vi "MQTT Session - Get Maximum QoS.vi"(0 "MQTT Session":T2, 7 "QoS":T1, 11 "error in":errorcluster) -> (4 "MQTT Session Out":T2, 8 "QoS":T1, 15 "error out":errorcluster)   [LabVIEW 2019, in "KoRE-MQTT.lvlib"]
doc: "Copyright (c) 2025 KoRElibs.com\nSPDX-License-Identifier: EUPL-1.2\n\nThis VI is licensed under the European Union Public License (EUPL) Version 1.2. You may use this VI unmodified in proprietary works. If you distribute a modified version of this file, the modified file must be released under the EUPL-1.2. Full license: https://joinup.ec.europa.eu/asset/eupl/eupl/1.2/"
uses:
  KoRE-MQTT.lvlib
  Public/TypeDefs/MQTT QoS Level.ctl
  Public/TypeDefs/MQTT Client Session.ctl
  TypeDefs/MQTT Client Session - Data Value Reference.ctl
  Public/TypeDefs/MQTT Client Session - Data.ctl
  Public/TypeDefs/MQTT Property - Will.ctl
  Public/TypeDefs/MQTT Property - CONNECT.ctl
  TypeDefs/MQTT Subscription - Info.ctl
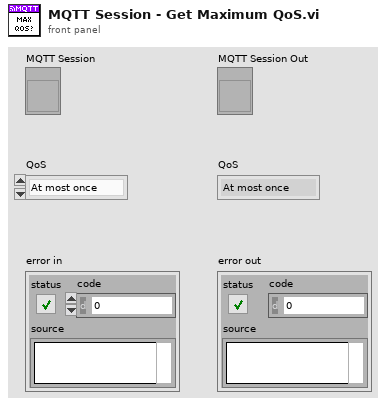
[diagram p1: front panel]
types:
  T1 = typedef "KoRE-MQTT.lvlib/MQTT QoS Level.ctl" = enum8{"At most once", "At least once", "Exactly once"}
  T2 = typedef "KoRE-MQTT.lvlib/MQTT Client Session.ctl" = refnum<vi>
  T3 = typedef "KoRE-MQTT.lvlib/MQTT Client Session - Data Value Reference.ctl" = refnum<data-value>
  T4 = typedef "KoRE-MQTT.lvlib/MQTT Client Session - Data.ctl" = cluster{"TCP ref":refnum<k5>, "Next Packet Id":u16, "Version":u8, "Host":string, "Port":u16, "Ping Delta":u32, "Username":string, "Password":string, "Will QoS":u8, "Will Retain":bool, "Will Topic":string, "Will Payload":string, "TCP Timeout":i32, "Semaphore":T5, "In-Flight Messages":variant, "Close":bool, "Last Send":u32, "Keep Alive":u16, "Last Ping RTT":u32, "Last Ping":u32, "Will Properties":T6[], "Session Expiry Interval":u32, "Maximum QoS":u8, "Retain Available":bool, "Server Maximum Packet Size":u32, "Client Identifier":string, "Server Topic Alias Maximum":u16, "Wildcard Subscription Available":bool, "Subscription Identifier Available":bool, "Shared Subscription Available":bool, "Connect Properties":T7[], "Client Maximum Packet Size":u32, "Client Topic Alias Maximum":u16, "Server Receive Maximum":u16, "Client Receive Maximum":u16, "TLS cfg":refnum<k36>, "Subscriptions":T8[]}
  T5 = typedef "Semaphore RefNum" = refnum<k1>
  T6 = typedef "KoRE-MQTT.lvlib/MQTT Property - Will.ctl" = cluster{"Property":u8, "Value":string}
  T7 = typedef "KoRE-MQTT.lvlib/MQTT Property - CONNECT.ctl" = cluster{"Property":u8, "Value":string}
  T8 = typedef "KoRE-MQTT.lvlib/MQTT Subscription - Info.ctl" = cluster{"Packet Id":u16, "Index":u16, "Identifier":u32, "QoS":u8, "Topic Filter":string, "Reason Code":u8, "Reason String":string, "Granted":bool}
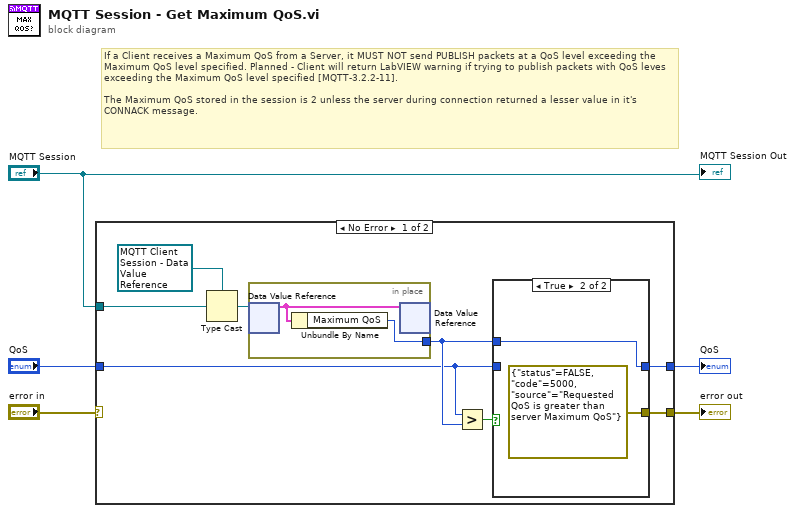
[diagram p0: block diagram]
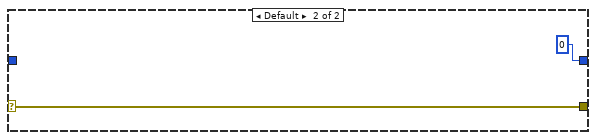
[diagram p3: hidden frame]
diagram:
  # "If a Client receives a Maximum QoS from a Server, it MUST NOT send PUBLISH packets at a QoS level exceeding the Maximum QoS level specified.\tPlanned - Client will return LabVIEW warning if trying to publish packets with QoS leves exceeding the Maximum QoS level specified [MQTT-3.2.2-11].\n\nThe Maximum QoS stored in the session is 2 unless the server during connection returned a lesser value in it's CONNACK message."
  n1 = case shown="No Error" "error in" {
    selector: "error in" -> [_ w20]
    tunnel: [w9 u8 0 ("Desired QoS")] -> w5
    tunnel: [w8 w20] -> w4
    tunnel: "QoS" -> [w7 _]
    tunnel: "MQTT Session" -> [w6 _]
    frame No Error {
      n2 = Type Cast(type=T3 refnum ("data value reference"), x=w6) -> (*(type *) &x=w12:T3)
      n3 = in-place {
        in-place-border: [w17] -> w10
        n4 = in-place-dvr #1(w12) -> (w18:T4)  [unwired: 1 out]
        n5 = Unbundle By Name(w18) -> ("Maximum QoS"=w17:u8)
        n6 = in-place-dvr #1(w18) -> ()  [unwired: 2 out]
      }
      n7 = Greater?(x=w7, y=w10) -> (0:w11:bool)
      n8 = case shown="True" w11 {
        tunnel: w10 -> [_ w16]
        tunnel: [w14 w16] -> w9
        tunnel: w7 -> [w14 _]
        tunnel: [_ errorcluster {"status"=FALSE, "code"=5000, "source"="Requested QoS is greater than server Maximum QoS"} ("error in")] -> w8
        frame False {
        }
        frame True {
        }
      }
    }
    frame Default {
    }
  }
  "QoS" <- w5
  "error out" <- w4
  "MQTT Session Out" <- "MQTT Session"
